vi "VIH ProjFile - Item Rule - Write.vi"(7 "Project Folder":path, 8 "error in":errorcluster, 9 "Item Rule":T1, 10 "Path":path, 11 "XML Parent Item":refnum<k20>) -> (0 "error out":errorcluster, 3 "dup XML Parent Item":refnum<k20>)   [LabVIEW 2014]
doc: "::: VI Helpeks :::\nCopyright (c) 2000-2026 Konstantin Shifershteyn. All rights reserved."
uses:
  _VIH HelpGen.llb/VIH HelpGen Typedef - Cluster - File Rule.ctl
  _VIH HelpGen.llb/VIH HelpGen Typedef - Enum - Default,Enable,Disable.ctl
  _VIH HelpGen.llb/VIH HelpGen Typedef - Cluster - File Rule - Source Paths.ctl
  _VIH HelpGen.llb/VIH HelpGen Typedef - Cluster - File Rule - Target Paths.ctl
  _VIH HelpGen.llb/VIH HelpGen Typedef - Enum - Description Mode.ctl
  _VIH HelpGen.llb/VIH HelpGen Typedef - Cluster - Control Rule.ctl
  _VIH HelpGen.llb/VIH HelpGen Typedef - Cluster - Enum Value Info.ctl
  _VIH HelpGen.llb/VIH HelpGen Typedef - Cluster - Group Rule - Flags.ctl
  <vilib>/xml/Close Reference(Node).vi
  <resource>/objmgr/DOMUserDefRef.rc
  <vilib>/xml/NI_XML.lvlib
panel:
  in  "Item Rule (data)":T1
  # "VI Helpeks\nCopyright (c) 2012-2026 Konstantin Shifershteyn"
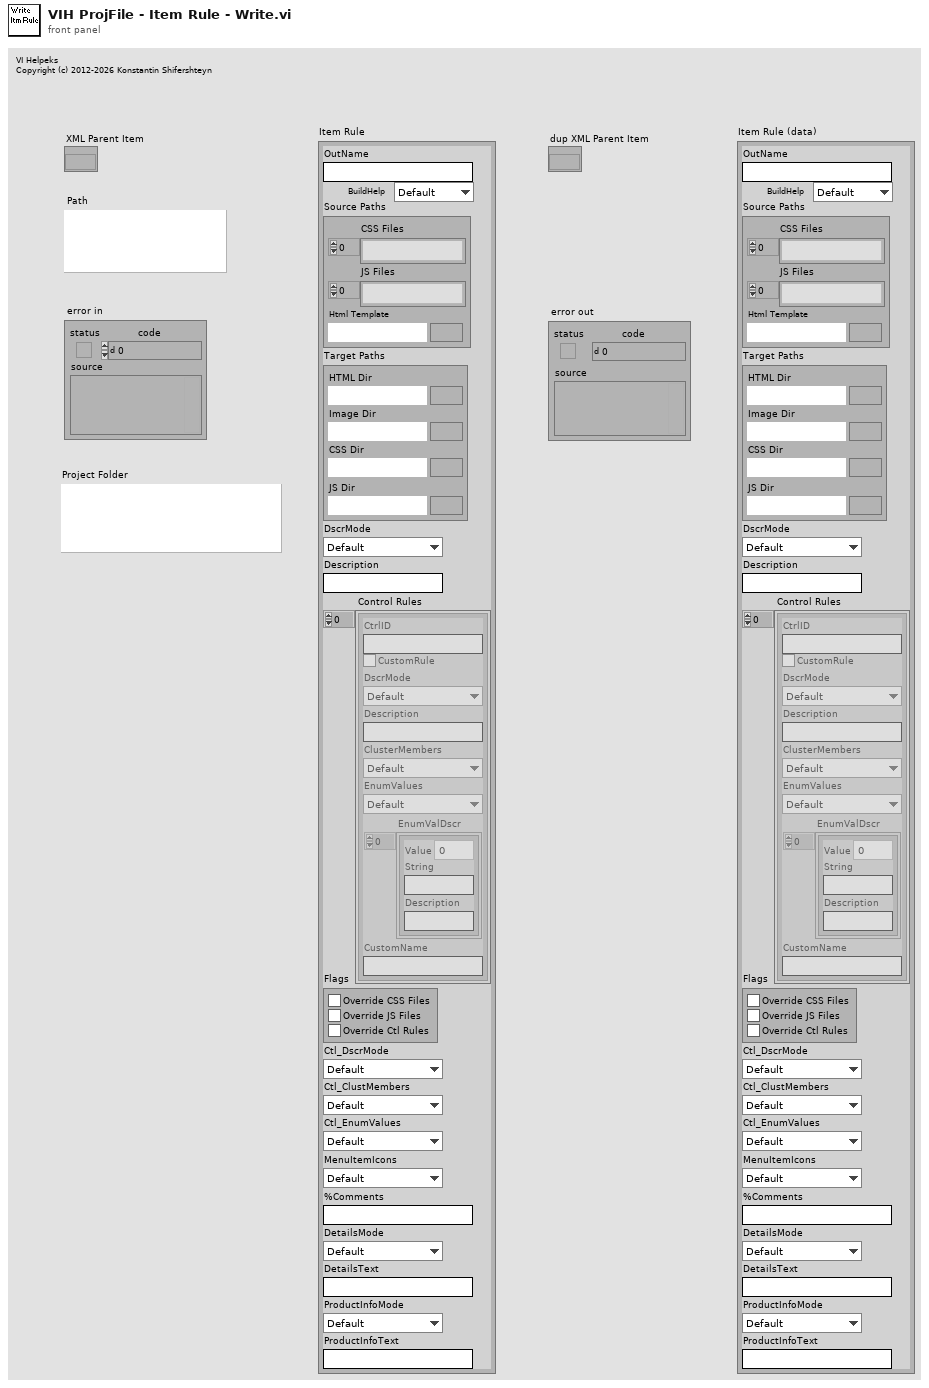
[diagram p1: front panel]
types:
  T1 = typedef "VIH HelpGen Typedef - Cluster - File Rule.ctl" = cluster{"OutName":string, "BuildHelp":T2, "Source Paths":T3, "Target Paths":T4, "DscrMode":T5, "Description":string, "Control Rules":T6[], "Flags":T8, "Ctl_DscrMode":T5, "Ctl_ClustMembers":T2, "Ctl_EnumValues":T2, "MenuItemIcons":T2, "%Comments":string, "DetailsMode":T5, "DetailsText":string, "ProductInfoMode":T2, "ProductInfoText":string}
  T2 = typedef "VIH HelpGen Typedef - Enum - Default,Enable,Disable.ctl" = enum16{"Default", "Enable", "Disable"}
  T3 = typedef "VIH HelpGen Typedef - Cluster - File Rule - Source Paths.ctl" = cluster{"CSS Files":path[], "JS Files":path[], "Html Template":path}
  T4 = typedef "VIH HelpGen Typedef - Cluster - File Rule - Target Paths.ctl" = cluster{"HTML Dir":path, "Image Dir":path, "CSS Dir":path, "JS Dir":path}
  T5 = typedef "VIH HelpGen Typedef - Enum - Description Mode.ctl" = enum16{"Default", "Description", "Description1", "Description2", "Custom", "None"}
  T6 = typedef "VIH HelpGen Typedef - Cluster - Control Rule.ctl" = cluster{"CtrlID":string, "CustomRule":bool, "DscrMode":T5, "Description":string, "ClusterMembers":T2, "EnumValues":T2, "EnumValDscr":T7[], "CustomName":string}
  T7 = typedef "VIH HelpGen Typedef - Cluster - Enum Value Info.ctl" = cluster{"Value":ext, "String":string, "Description":string}
  T8 = typedef "VIH HelpGen Typedef - Cluster - Group Rule - Flags.ctl" = cluster{"Override CSS Files":bool, "Override JS Files":bool, "Override Ctl Rules":bool}
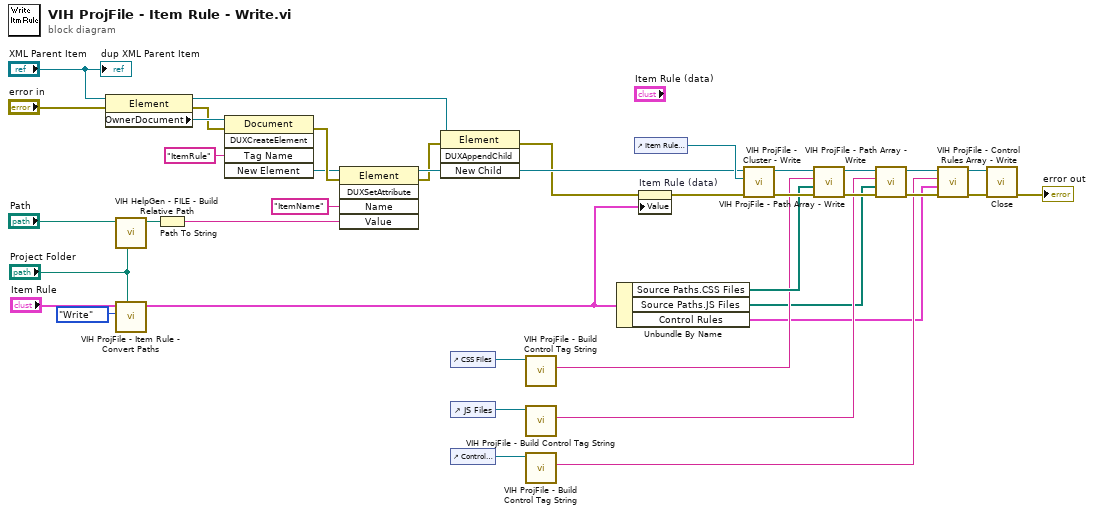
[diagram p0: block diagram]
diagram:
  n1 = property class="Element"(reference="XML Parent Item", error in="error in") -> (reference out=w10:refnum<k20>, error out=w8:errorcluster, "OwnerDocument"=w11:refnum<k20>)
  n2 = call "VIH HelpGen - FILE - Build Relative Path.vi"("Root Path"="Project Folder", "Path in"="Path") -> ("Path out"=w4:path)  [unwired: 9 in]
  n3 = call "VIH ProjFile - Item Rule - Convert Paths.vi"("Root Dir"="Project Folder", "Operation"=enum16{"Read", "Write"}."Write", "Item Rule"="Item Rule") -> ("Item Rule out"=w6:T1)  [unwired: 8 in]
  n4 = Path To String(path=w4) -> (string=w2:string)
  n5 = invoke class="Document" method="DUXCreateElement"(reference=w11, error in=w8, "Tag Name"="ItemRule") -> (error out=w18:errorcluster, "New Element"=w17:refnum<k20>)  [unwired: 2 in, 3 out]
  n6 = invoke class="Element" method="DUXSetAttribute"(reference=w17, error in=w18, "Name"="ItemName", "Value"=w2) -> (reference out=w38:refnum<k20>, error out=w14:errorcluster)  [unwired: 1 in, 3 out]
  n7 = invoke class="Element" method="DUXAppendChild"(reference=w10, error in=w14, "New Child"=w38) -> (error out=w36:errorcluster)  [unwired: 1 in, 3 out]
  n8 = control-ref of="CSS Files"() -> (w19:refnum<vi>)
  n9 = control-ref of="JS Files"() -> (w20:refnum<vi>)
  n10 = control-ref of="Control Rules"() -> (w13:refnum<vi>)
  n11 = call "VIH ProjFile - Build Control Tag String.vi"("Ctl Refnum"=w19) -> ("Control Tag"=w31:string)  [unwired: 6 in, 4 out]
  n12 = call "VIH ProjFile - Build Control Tag String.vi"("Ctl Refnum"=w20) -> ("Control Tag"=w28:string)  [unwired: 6 in, 4 out]
  n13 = call "VIH ProjFile - Build Control Tag String.vi"("Ctl Refnum"=w13) -> ("Control Tag"=w22:string)  [unwired: 6 in, 4 out]
  n14 = Unbundle By Name(w6) -> ("Source Paths.CSS Files"=w32:path[], "Source Paths.JS Files"=w27:path[], "Control Rules"=w21:T6[])
  n15 = control-ref of="Item Rule (data)"() -> (w39:refnum<vi>)
  n16 = property on="Item Rule (data)" class="Clust (strict)"(error in=w36, "Value"=w6) -> (error out=w37:errorcluster)  [unwired: 1 in, 1 out]
  n17 = call "VIH ProjFile - Cluster - Write.vi"("error in"=w37, "Ctl Refnum"=w39, "XML Parent Item"=w38) -> ("error out"=w33:errorcluster, "dup XML Parent Item"=w34:refnum<k20>)  [unwired: 7 in]
  n18 = call "VIH ProjFile - Path Array - Write.vi"("error in"=w33, "Paths"=w32, "Property Name"=w31, "XML Parent Item"=w34) -> ("error out"=w29:errorcluster, "dup XML Parent Item"=w30:refnum<k20>)  [unwired: 6 in]
  n19 = call "VIH ProjFile - Path Array - Write.vi"("error in"=w29, "Paths"=w27, "Property Name"=w28, "XML Parent Item"=w30) -> ("error out"=w25:errorcluster, "dup XML Parent Item"=w26:refnum<k20>)  [unwired: 6 in]
  n20 = call "VIH ProjFile - Control Rules Array - Write.vi"("error in"=w25, "Control Rules"=w21, "Property Name"=w22, "XML Parent Item"=w26) -> ("error out"=w24:errorcluster, "dup XML Parent Item"=w23:refnum<k20>)  [unwired: 6 in]
  n21 = call-poly <vilib>:"Close.vi"("error in (no error)"=w24, "node"=w23) -> ("error out"=→"error out":errorcluster)  [unwired: 7 in]
  "dup XML Parent Item" <- "XML Parent Item"
